vi "GpuMat Download_Image.vi"(8 "error in (no error)":errorcluster, 10 "Dst":T1, 11 "GpuMat in":refnum<class "GpuMat.lvclass">) -> (0 "error out":errorcluster, 2 "Dst out":T1, 3 "GpuMat out":refnum<class "GpuMat.lvclass">)   [LabVIEW 2020, in "OpenLvVision_OpenCv.lvlib" / "Cuda.lvlib" / "GpuMat.lvclass"]
doc: "Downloads processed data from the GPU matrix directly into a Image."
uses:
  GpuMat.lvclass
  C:/Users/lukas/Documents/OpenLvVision_OpenCv/SourceCode/LabView/OpenLvVision_OpenCv/_LvHelpers/EdvrObject/EdvrObject.lvclass
  <vilib>/vision/Image Controls.llb/IMAQ Image.ctl
  _LvHelpers/EdvrObject/EdvrObject.lvclass/EdvrObject.ctl
  <vilib>/Utility/error.llb/Error Cluster From Error Code.vi
  _LvHelpers/MatHandling/RegisterMat/RegisterMat_Image.vi
  _LvHelpers/MatHandling/UnregisterMat/UnregisterMat_Image.vi
  OpenLvVision_OpenCv.lvlib
  _LvHelpers/EdvrObject/EdvrObject.lvclass
  <vilib>/OpenLvVision/OpenLvVision_Image/Management/OLV Management.lvlib
  <vilib>/ErrorRing/Error Ring.xnode
  Dlls/OlvOpenCvWrapper.dll
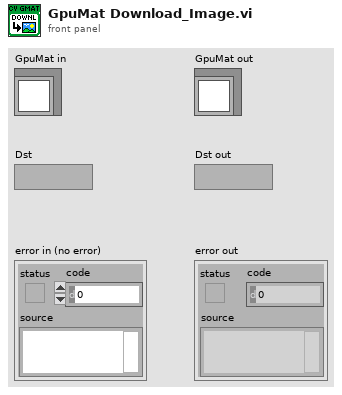
[diagram p1: front panel]
types:
  T1 = typedef "IMAQ Image.ctl" = refnum<image>
  T2 = typedef "OpenLvVision_OpenCv.lvlib/GpuMatInfo.ctl" = cluster{"Rows":i32, "Cols":i32, "cvType":T3, "Channels":i32, "depth":i32}
  T3 = typedef "OpenLvVision_OpenCv.lvlib/cvType.ctl" = enum32{"CV_8UC1", "CV_8SC1", "CV_16UC1", "CV_16SC1", "CV_32SC1", "CV_32FC1", "CV_64FC1", "CV_16FC1", "CV_8UC2", "CV_8SC2", "CV_16UC2", "CV_16SC2", "CV_32SC2", "CV_32FC2", "CV_64FC2", "CV_16FC2", "CV_8UC3", "CV_8SC3", "CV_16UC3", "CV_16SC3", "CV_32SC3", "CV_32FC3", "CV_64FC3", "CV_16FC3", "CV_8UC4", "CV_8SC4", "CV_16UC4", "CV_16SC4", "CV_32SC4", "CV_32FC4", "CV_64FC4", "CV_16FC4"}
  T4 = typedef "OLV OpenLvVision_Image.lvlib/OLV Management.lvlib/OLV Image.ctl" = refnum<image>
  T5 = typedef "OLV OpenLvVision_Image.lvlib/OLV Management.lvlib/OLV ImageType.ctl" = enum16{"Mono U8", "Mono U16", "Mono I16", "Mono SGL", "Color U32", "Color U64", "Complex CSG"}
  T6 = typedef "OpenLvVision_OpenCv.lvlib/MatInfo.ctl" = cluster{"Datatype":T7, "Height":i32, "Width":i32, "Channels":i32, "LineWidth":i32, "Null":u8}
  T7 = typedef "OpenLvVision_OpenCv.lvlib/LvDatatype.ctl" = enum32{"Undefined", "U8", "I8", "U16", "I16", "U32_Color", "I32", "U64_Color", "I64", "SGL", "DBL", "Complex SGL", "Complex DBL", "Array 1D U8", "Array 1D I8", "Array 1D U16", "Array 1D I16", "Array 1D U32_Color", "Array 1D I32", "Array 1D U64_Color", "Array 1D I64", "Array 1D SGL", "Array 1D DBL", "Array 1D Complex SGL", "Array 1D Complex DBL", "Array 2D U8", "Array 2D I8", "Array 2D U16", "Array 2D I16", "Array 2D U32", "Array 2D U32_Color", "Array 2D I32", "Array 2D U64", "Array 2D U64_Color", "Array 2D I64", "Array 2D SGL", "Array 2D DBL", "Array 2D Complex SGL", "Array 2D Complex DBL", "Image Mono U8", "Image Mono U16", "Image Mono I16", "Image Mono SGL", "Image Color U32", "Image Color U64", "ImageComplex Sgl", "Array1d_2dPointI32", "Array1d_2dPointSGL", "Array1d_2dPointDBL", "Array1d_3dPointI32", "Array1d_3dPointSGL", "Array1d_3dPointDBL", "Array1d_4dPointI32", "Array1d_4dPointSGL", "Array1d_4dPointDBL", "ArrayNchwU8", "ArrayNchwI8", "ArrayNchwU16", "ArrayNchwI16", "ArrayNchwU32_Color", "ArrayNchwI32", "ArrayNchwU64_Color", "ArrayNchwSgl", "ArrayNchwDbl", "ArrayNchwComplexSgl", "ArrayNchwComplexDbl"}
  T8 = typedef "OpenLvVision_OpenCv.lvlib/EdvrObject.lvclass/Edvr.ctl" = refnum<data-value>
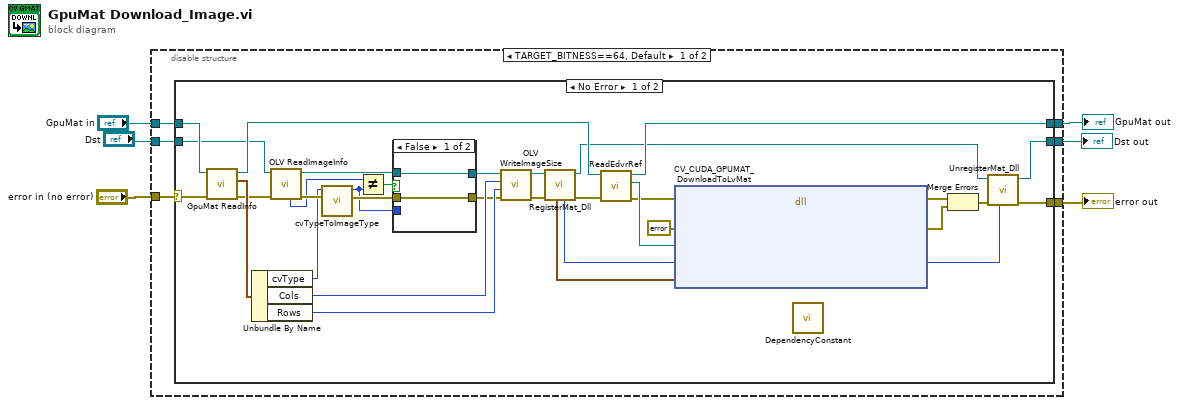
[diagram p0: block diagram]
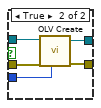
[diagram p2: hidden frame]
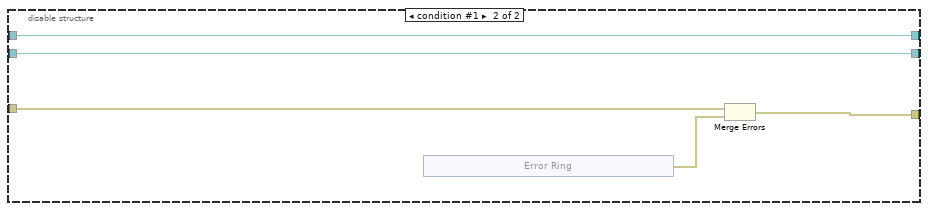
[diagram p4: hidden frame]
diagram:
  n1 = disable-structure shown="TARGET_BITNESS==64, Default" {
    disable-tunnel: "error in (no error)" -> [w12 w59]
    disable-tunnel: [w11 w60] -> w3
    disable-tunnel: "GpuMat in" -> [w10 w56]
    disable-tunnel: [w9 w56] -> w1
    disable-tunnel: [w8 w57] -> w2
    disable-tunnel: "Dst" -> [w7 w57]
    frame condition #0 (active) {
      n2 = case shown="No Error" w12 {
        selector: w12 -> [w14 w55]
        tunnel: [w36 w55] -> w11
        tunnel: w10 -> [w40 w54]
        tunnel: [w41 w54] -> w9
        tunnel: [w37 w53] -> w8
        tunnel: w7 -> [w25 w53]
        frame No Error {
          n3 = call "GpuMat ReadInfo.vi"("error in (no error)"=w14, "GpuMat in"=w40) -> ("error out"=w26:errorcluster, "GpuMatInfo"=w32:T2, "GpuMat out"=w39:refnum<class "GpuMat.lvclass">)  [unwired: 7 in]
          n4 = Unbundle By Name(w32) -> ("cvType"=w21:T3, "Cols"=w31:i32, "Rows"=w30:i32)
          n5 = call <vilib>:"OLV ReadImageInfo.vi"("error in"=w26, "Image Reference In"=w25) -> ("error out"=w24:errorcluster, "Image Reference Out"=w22:T4, "Image Type"=w19:T5)  [unwired: 4 in, 3 out]
          n6 = call "cvTypeToImageType.vi"("error in"=w24, "cvType"=w21) -> ("error out"=w23:errorcluster, "Image Type"=w16:T5)  [unwired: 8 in]
          n7 = Not Equal?(x=w19, y=w16) -> (x != y?=w20:bool)
          n8 = case shown="False" w20 {
            tunnel: w23 -> [w47 w52]
            tunnel: w22 -> [w46 w50]
            tunnel: [w47 w51] -> w18
            tunnel: [w46 w49] -> w17
            tunnel: w16 -> [_ w48]
            frame False {
            }
            frame True {
              n9 = call <vilib>:"OLV Create.vi"("Image Type"=w48, "error in"=w52, "Image Name"=w50) -> ("error out"=w51:errorcluster, "Image Reference Out"=w49:T4)  [unwired: 7 in]
            }
          }
          n10 = call <vilib>:"OLV WriteImageSize.vi"("error in"=w18, "Height"=w30, "Width"=w31, "Image Reference In"=w17) -> ("error out"=w29:errorcluster, "Image Reference Out"=w28:T4)  [unwired: 6 in]
          n11 = call-poly "RegisterMat_Dll.vi"("error in"=w29, "Image Reference In"=w28) -> ("error out"=w38:errorcluster, "Image Reference Out"=w27:T4, "AdressOrData"=w35:u64, "Mat"=w34:T6)  [unwired: 6 in]
          n12 = call "ReadEdvrRef.vi"("error in (no error)"=w38, "EdvrObject in"=w39) -> ("error out"=w15:errorcluster, "Edvr"=w42:T8, "EdvrObject out"=w41:refnum<class "GpuMat.lvclass">)  [unwired: 7 in]
          n13 = dll-call lib="C:/Users/lukas/Documents/OpenLvVision_OpenCv/SourceCode/LabView/OpenLvVision_OpenCv/Dlls/OlvOpenCvWrapper.dll" fn="CV_CUDA_GPUMAT_DownloadToLvMat"(error in=w15, "Error"=errorcluster {"status"=FALSE, "code"=0, "source"=""} ("error out"), "edvrRef"=w42, "addressDst"=w35, "matInfoDst"=w34) -> (error out=w45:errorcluster, "Error"=w44:errorcluster, "addressDst"=w33:u64)  [unwired: 5 in, 1 out]
          n14 = call "DependencyConstant.vi"() -> ()  [unwired: 12 in]
          n15 = Merge Errors(w45, w44) -> (w13:errorcluster)
          n16 = call-poly "UnregisterMat_Dll.vi"("AdressOrData"=w33, "error in"=w13, "Image Reference In"=w27) -> ("error out"=w36:errorcluster, "Image Reference Out"=w37:T4)  [unwired: 7 in]
        }
        frame Error {
        }
      }
    }
    frame condition #1 {
      n17 = xnode "Error Ring"() -> ("error out"=w58:errorcluster)
      n18 = Merge Errors(w59, w58) -> (w60:errorcluster)
    }
  }
  "error out" <- w3
  "GpuMat out" <- w1
  "Dst out" <- w2
